vi "Test Raw PubSub.vi"() -> ()   [LabVIEW 2021]
uses:
  typedef/Publisher Configuration.ctl
  typedef/Subscriber Configuration.ctl
  typedef/Publisher Info.ctl
  f88eec82-93b0-4b73-b241-8ea333a750c0.vi
  3ba9bed8-dd13-4a10-92c8-30b1fa84fb7c.vi
  06d7ed46-2aa9-4a58-a146-244b7cae5bd9.vi
  009ccb22-fdf8-4a9a-a05b-4c49a602eecd.vi
  336a4bb3-c987-4874-ab49-fbc20b376376.vi
  d958d2fb-f6ac-4309-8ce0-3eafaa81bea2.vi
  75a58427-ab38-4537-8b56-a141a3672aa3.vi
  6786380f-354a-4568-8806-a035e3271ed9.vi
  422841d8-307b-4ec0-b2db-fbf3b15355db.vi
  2722b832-a6ed-40a1-94d0-5438662527b8.vi
  4f573ed8-5eea-442c-8954-fd33649ad94d.vi
  96719cce-9db7-4fd0-8c85-b901c094f5f7.vi
  9c36c4f5-fd14-474a-8537-d667d986c500.vi
  37cd7a68-2c72-48bd-8358-2e5ff7ad5fbf.vi
  25405cc9-b883-4350-b671-2b1f334a3515.vi
  af1225cd-10e8-4ded-be35-c9aec92c40b2.vi
  a487f0d3-ed83-4ff6-b1b9-975fbbcad064.vi
  1e4a52af-b425-4bd5-8079-be6529fa9e9c.vi
  d9d8694a-5329-4e50-a2e7-87effcffdca9.vi
  4327a0ae-2f84-4360-8cf5-e48e8584a04f.vi
  8254caa6-6f2b-4011-9217-4a5e3ed42d89.vi
  19e9252e-2146-4d1e-ba58-cc4f3a3c56cb.vi
  863d4d22-9275-487b-b92e-4ed484f7a1b3.vi
  c0f4674b-d7d9-47c2-9242-89a7410a619c.vi
  919f7c05-3ba9-40da-9afe-90bc52095352.vi
  1a02b84e-e0dd-4555-bba6-db125e571599.vi
  b1950baf-a6de-4c07-b8a3-a72aac12c1c1.vi
  ae4bf491-c0b7-44fa-a4a7-8158168e9fc6.vi
  ed865d3e-ab37-4a94-9a8c-dd2836983b09.vi
  5089277c-e4c2-417d-bf61-c3bd261b64ad.vi
  2648f811-d11d-4cf1-8e69-7cf28aed7662.vi
  4d02bc77-4783-49f2-a635-9fdf52d75067.vi
  6650dd4f-c820-41cd-8769-445f0eb68481.vi
  363597ae-3dcd-42a2-ad25-38ce26843048.vi
  43a2abd8-1115-4a6b-bb2f-cda109865661.vi
  76c65e38-25cb-4c5d-9514-de54a11eb46c.vi
  076b9f91-9c98-45bc-8a99-05568dd34c74.vi
  da7c517f-bb6b-476f-8057-eaeaf84c1734.vi
  75a22d6a-3c1f-452c-a0ab-9f852fbcf576.vi
  d28d170c-9ca3-4356-a02f-9b2902eae1eb.vi
  458cc294-3f79-4518-a0de-1932c661e4d9.vi
  4369ee51-5961-4433-b656-85aa5b427ae6.vi
  cfff3f0f-7213-4192-9fc9-75e3c3355763.vi
  39bd5219-0461-483e-bfc5-6ac24da31237.vi
  c31ef992-ca3f-413b-a618-0d329516adf2.vi
  e3428d73-0891-455a-b634-5f02aa550c64.vi
  c128d40d-42b3-4721-be74-df15ce752ec7.vi
  SubVIs/Get Path.vi
  SubVIs/Convert Error.vi
  f88eec82-93b0-4b73-b241-8ea333a750c0.vi/f164bb55-fadc-406a-97d8-e3295a396b46.vi
  SubVIs/Add Error.vi
  Refnum/Raw Publisher to Refnum.vi
  <vilib>/CIF Foundation/CIF Utilities/File/File/File Not Found Error Update.vi
  3ba9bed8-dd13-4a10-92c8-30b1fa84fb7c.vi/15451e88-64ef-462d-9cc0-58968935b893.vi
  Refnum/Raw Subscriber to Refnum.vi
  Refnum/Raw Publisher from Refnum.vi
  Refnum/Raw Subscriber from Refnum.vi
  336a4bb3-c987-4874-ab49-fbc20b376376.vi/f164bb55-fadc-406a-97d8-e3295a396b46.vi
  d958d2fb-f6ac-4309-8ce0-3eafaa81bea2.vi/15451e88-64ef-462d-9cc0-58968935b893.vi
  75a58427-ab38-4537-8b56-a141a3672aa3.vi/15451e88-64ef-462d-9cc0-58968935b893.vi
  4f573ed8-5eea-442c-8954-fd33649ad94d.vi/f164bb55-fadc-406a-97d8-e3295a396b46.vi
  96719cce-9db7-4fd0-8c85-b901c094f5f7.vi/15451e88-64ef-462d-9cc0-58968935b893.vi
  9c36c4f5-fd14-474a-8537-d667d986c500.vi/15451e88-64ef-462d-9cc0-58968935b893.vi
  a487f0d3-ed83-4ff6-b1b9-975fbbcad064.vi/f164bb55-fadc-406a-97d8-e3295a396b46.vi
  1e4a52af-b425-4bd5-8079-be6529fa9e9c.vi/15451e88-64ef-462d-9cc0-58968935b893.vi
  d9d8694a-5329-4e50-a2e7-87effcffdca9.vi/15451e88-64ef-462d-9cc0-58968935b893.vi
  863d4d22-9275-487b-b92e-4ed484f7a1b3.vi/f164bb55-fadc-406a-97d8-e3295a396b46.vi
  c0f4674b-d7d9-47c2-9242-89a7410a619c.vi/15451e88-64ef-462d-9cc0-58968935b893.vi
  919f7c05-3ba9-40da-9afe-90bc52095352.vi/15451e88-64ef-462d-9cc0-58968935b893.vi
  1a02b84e-e0dd-4555-bba6-db125e571599.vi/f164bb55-fadc-406a-97d8-e3295a396b46.vi
  ae4bf491-c0b7-44fa-a4a7-8158168e9fc6.vi/15451e88-64ef-462d-9cc0-58968935b893.vi
  5089277c-e4c2-417d-bf61-c3bd261b64ad.vi/f164bb55-fadc-406a-97d8-e3295a396b46.vi
  4d02bc77-4783-49f2-a635-9fdf52d75067.vi/15451e88-64ef-462d-9cc0-58968935b893.vi
  43a2abd8-1115-4a6b-bb2f-cda109865661.vi/f164bb55-fadc-406a-97d8-e3295a396b46.vi
  76c65e38-25cb-4c5d-9514-de54a11eb46c.vi/15451e88-64ef-462d-9cc0-58968935b893.vi
  458cc294-3f79-4518-a0de-1932c661e4d9.vi/f164bb55-fadc-406a-97d8-e3295a396b46.vi
  4369ee51-5961-4433-b656-85aa5b427ae6.vi/15451e88-64ef-462d-9cc0-58968935b893.vi
  c128d40d-42b3-4721-be74-df15ce752ec7.vi/f164bb55-fadc-406a-97d8-e3295a396b46.vi
  <vilib>/Utility/error.llb/Trim Whitespace.vi
  SubVIs/Add Error Core.vi
  <vilib>/CIF Foundation/CIF Utilities/DataTypes/Utilities/Get Element Info of Variant.vi
  SubVIs/Get Type String.vi
  <vilib>/CIF Foundation/CIF Utilities/DataTypes/Utilities/Get JSON Descriptor of Variant.vi
  SubVIs/Convert Error Core.vi
  <vilib>/CIF Foundation/CIF Utilities/File/SubVIs/File Not Found Error Core.vi
  Iceoryx.lvlib
panel:
  out "status":string
  out "pass":bool
  out "error out":errorcluster
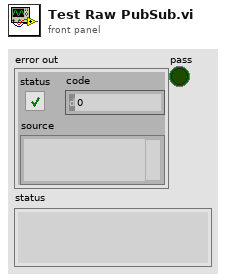
[diagram p1: front panel]
types:
  T1 = typedef "Iceoryx.lvlib/Subscriber Configuration.ctl" = cluster{"Name":string, "Topic":string, "Type":string, "Backpressure":bool}
  T2 = typedef "Iceoryx.lvlib/Publisher Configuration.ctl" = cluster{"Name":string, "Topic":string, "Type":string, "Best Effort Subscribers":u32, "Backpressure Subscribers":u32, "Best Effort Queue Depth":u32, "Backpressure Queue Depth":u32}
  T3 = typedef "Iceoryx.lvlib/Publisher Info.ctl" = cluster{"Type":string, "Element Size":u32, "Max Elements in Array":u32, "Backpressure Queue Depth":u32, "Best Effort Queue Depth":u32}
  T4 = typedef "Iceoryx.lvlib/Raw Publisher Refnum.ctl" = cluster{"refnum":u64, "Raw Pub":enum8{"rawpub"}}
  T5 = typedef "Iceoryx.lvlib/Raw Subscriber Refnum.ctl" = cluster{"refnum":u64, "Raw Sub":enum8{"rawsub"}}
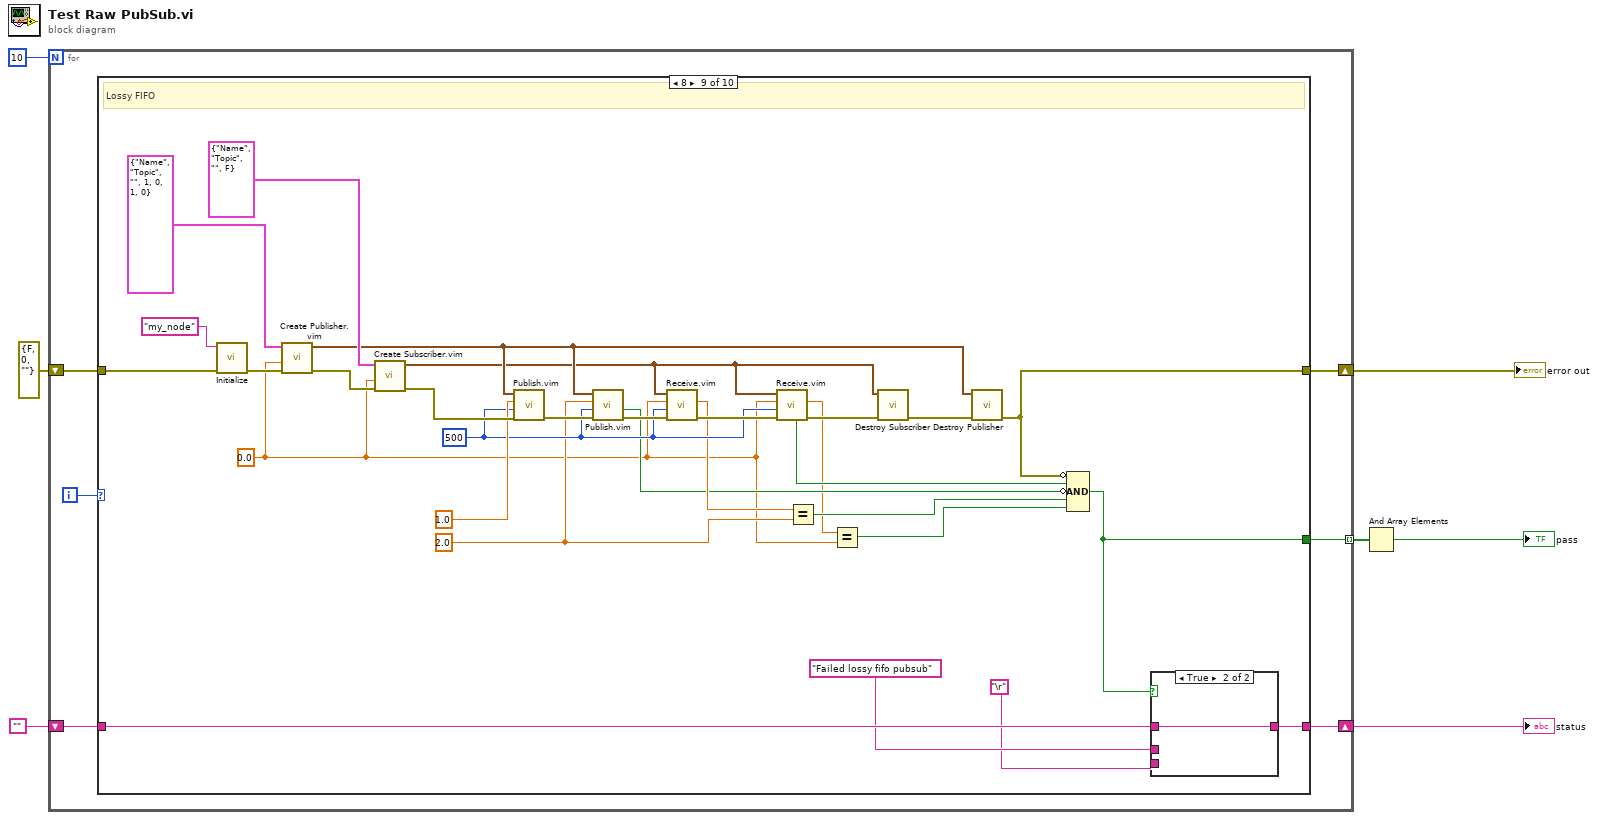
[diagram p0: block diagram]
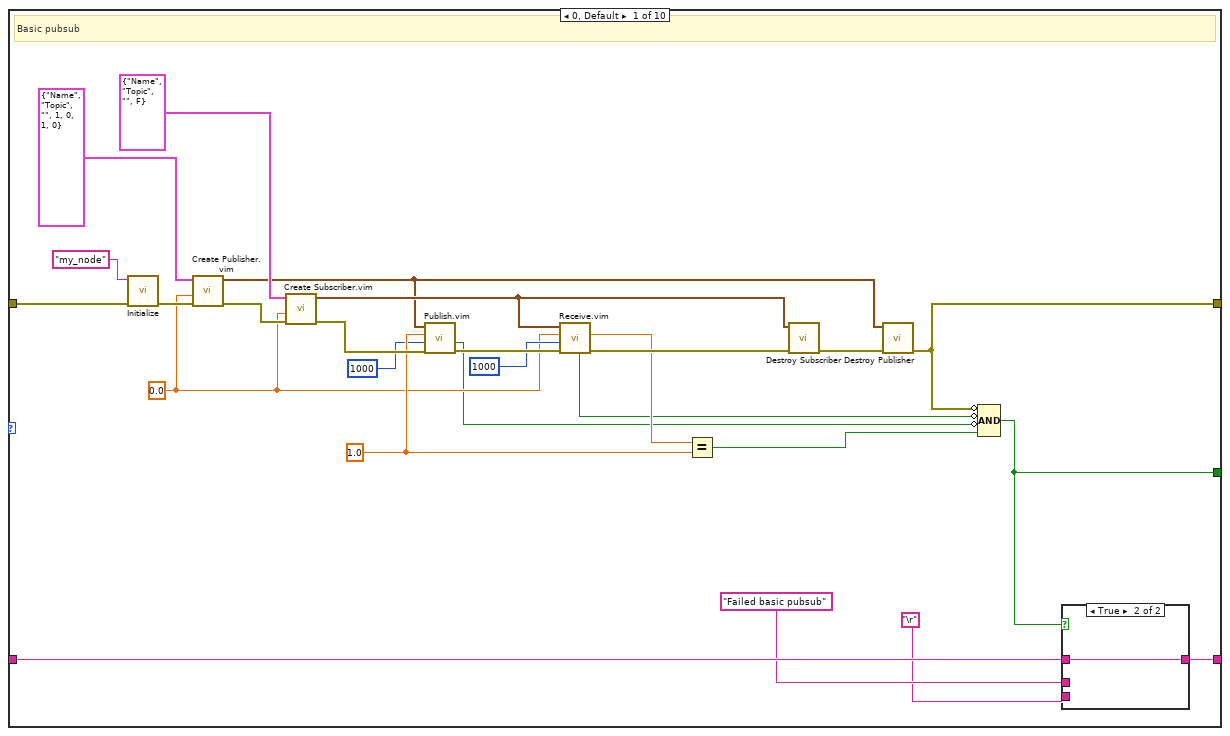
[diagram p2: hidden frame]
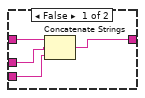
[diagram p3: hidden frame]
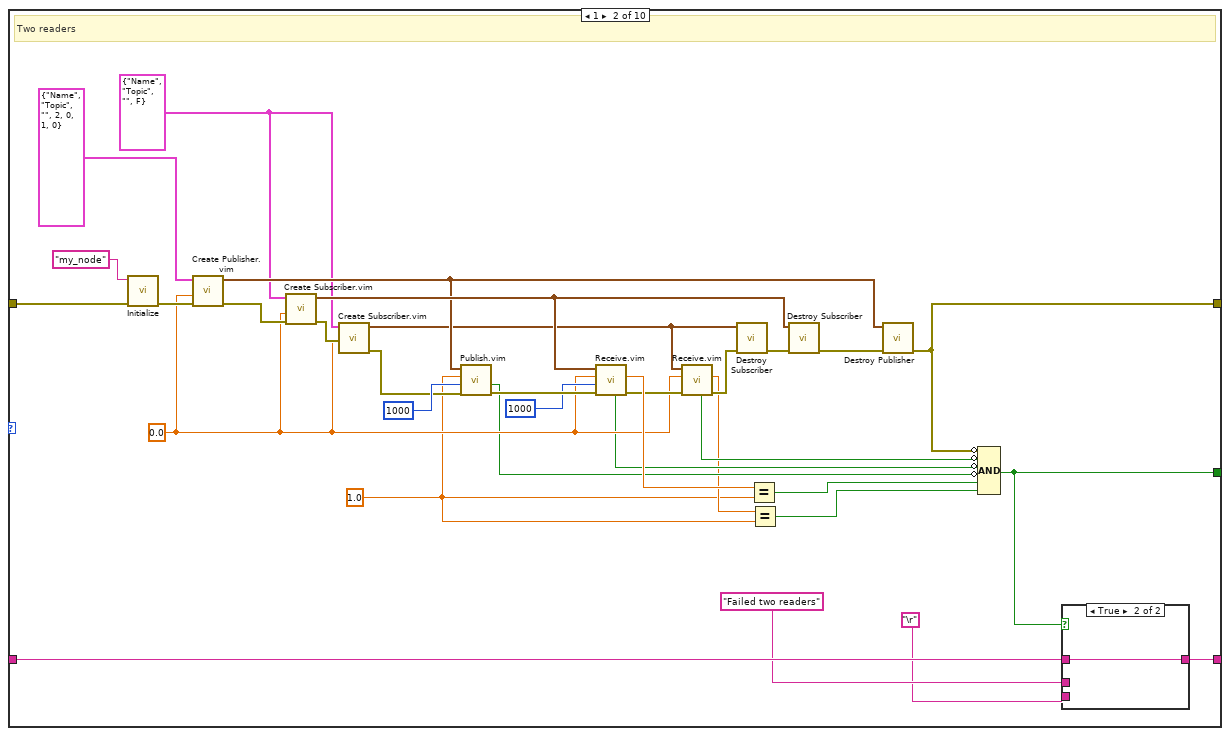
[diagram p4: hidden frame]
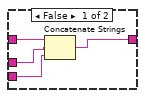
[diagram p5: hidden frame]
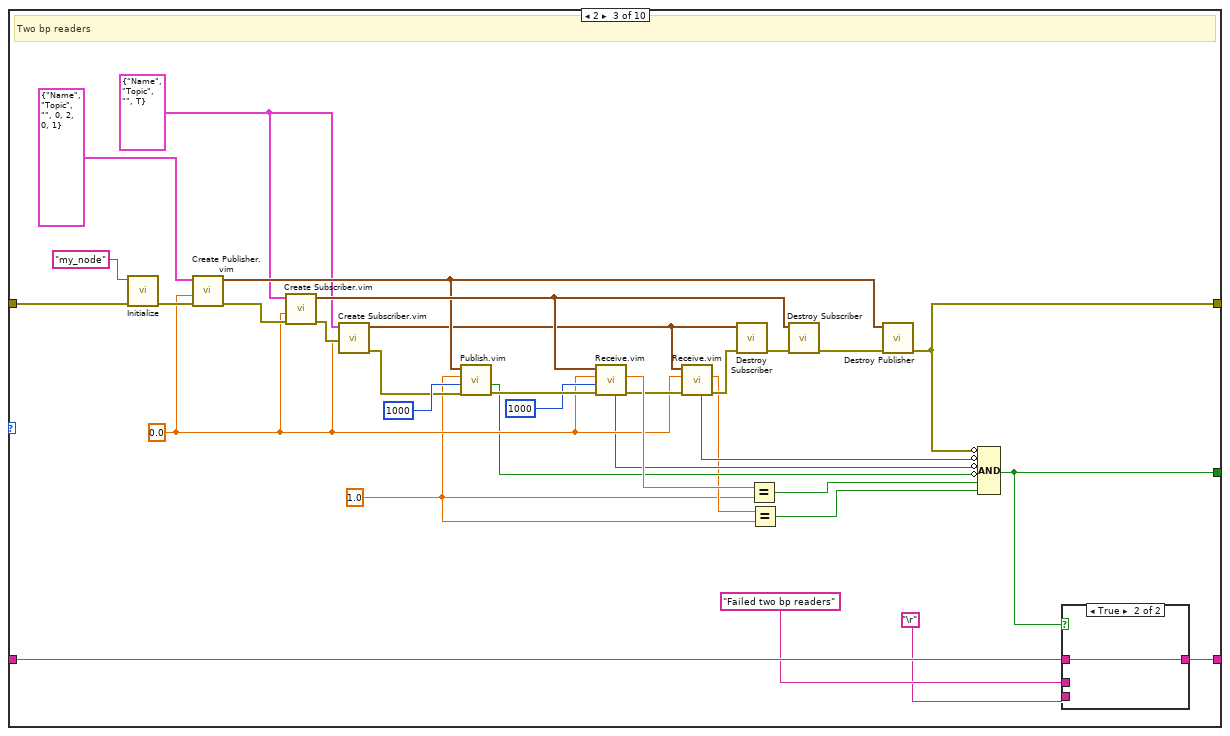
[diagram p6: hidden frame]
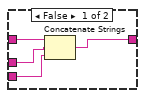
[diagram p7: hidden frame]
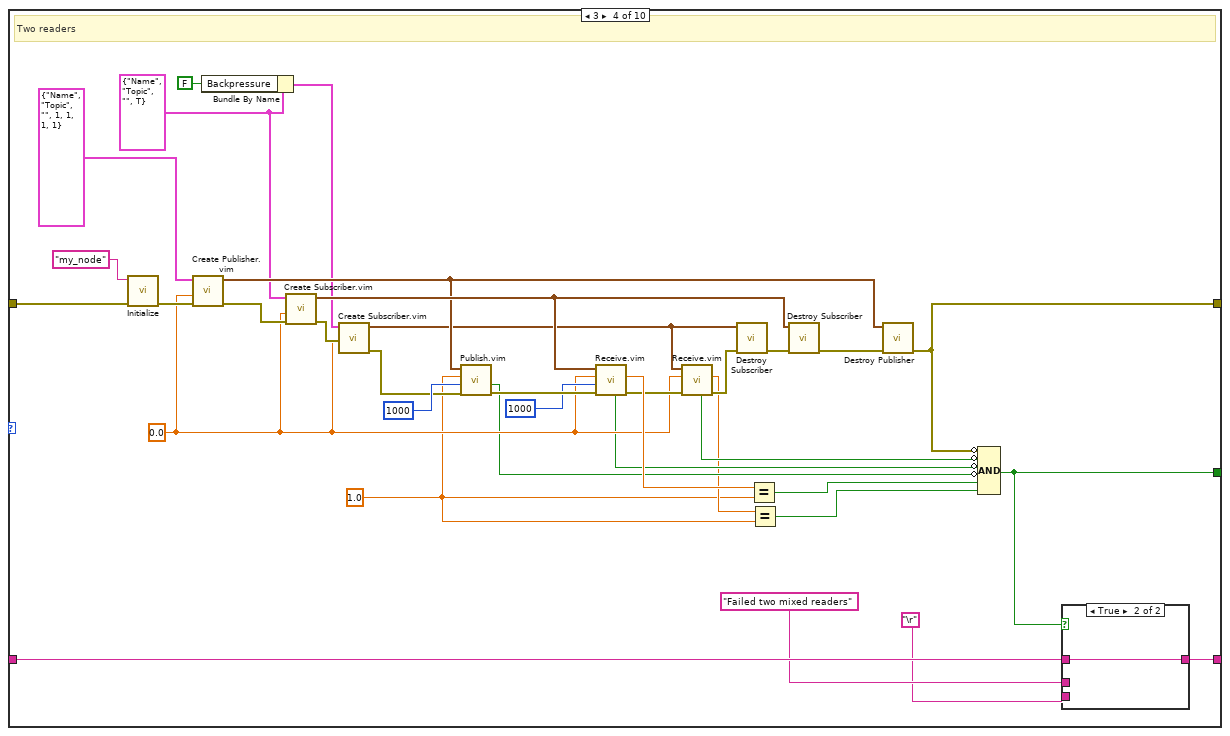
[diagram p8: hidden frame]
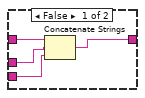
[diagram p9: hidden frame]
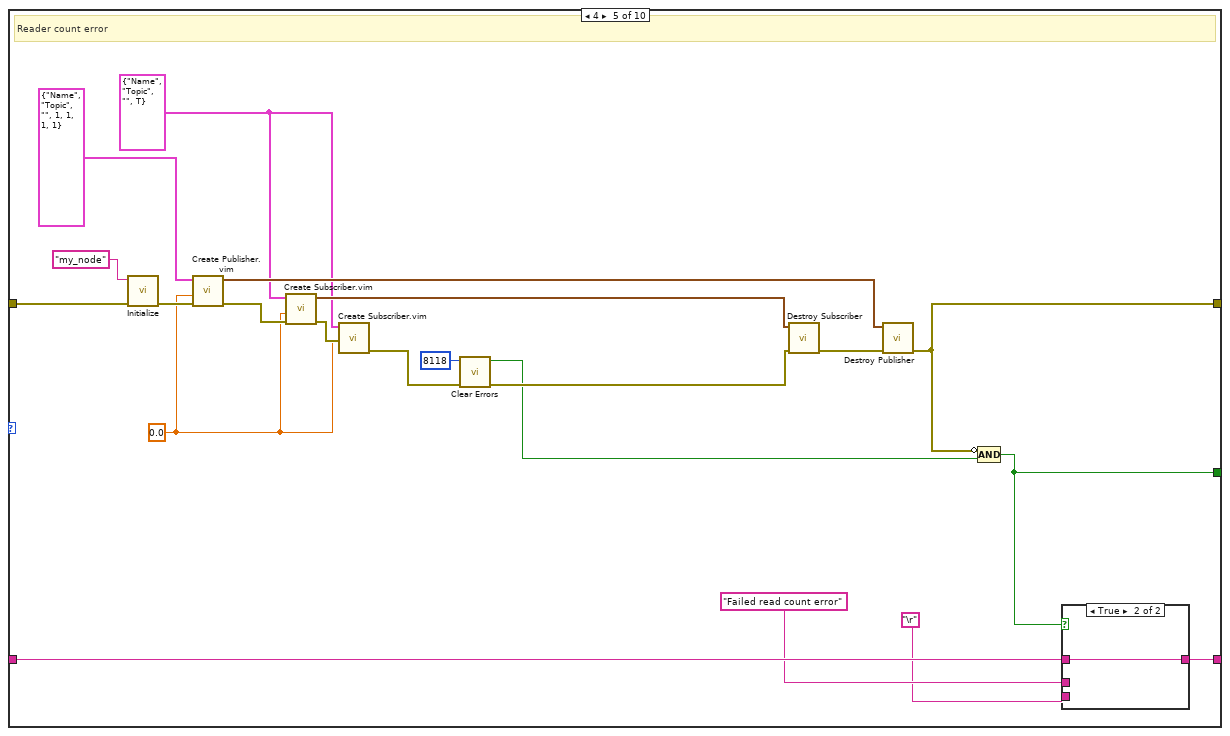
[diagram p10: hidden frame]
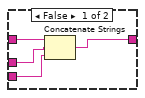
[diagram p11: hidden frame]
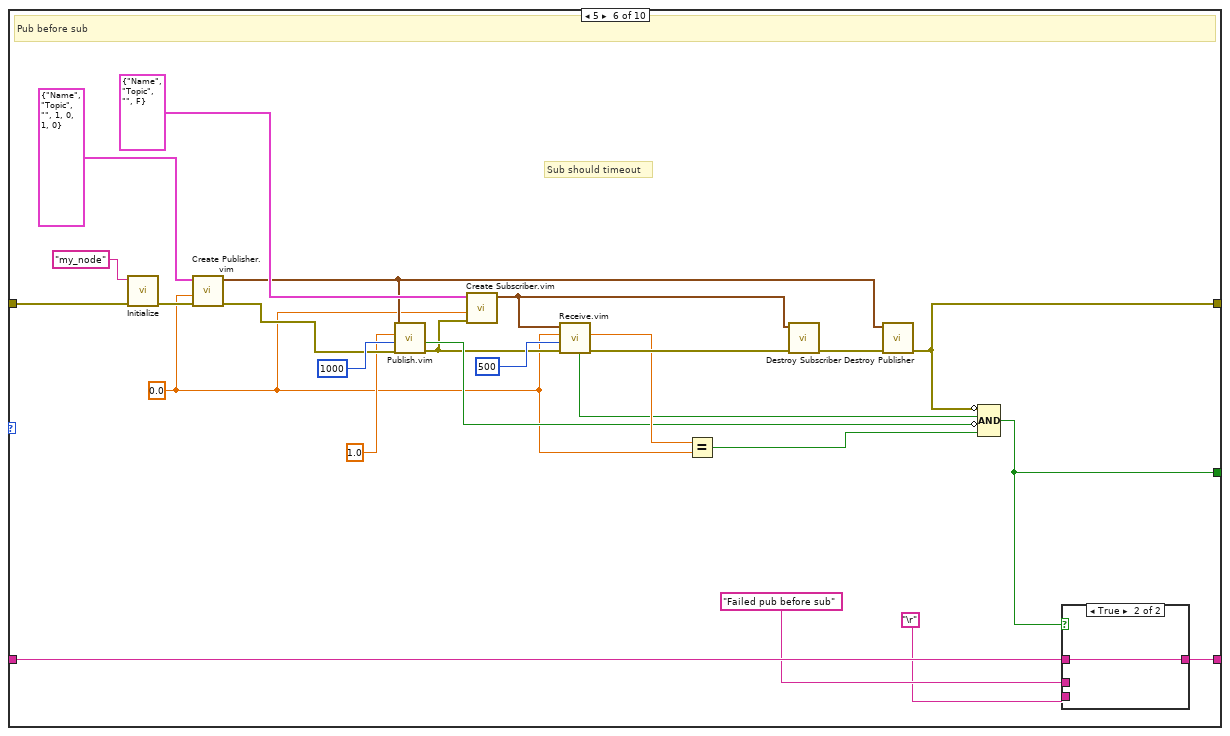
[diagram p12: hidden frame]
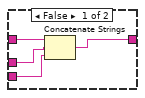
[diagram p13: hidden frame]
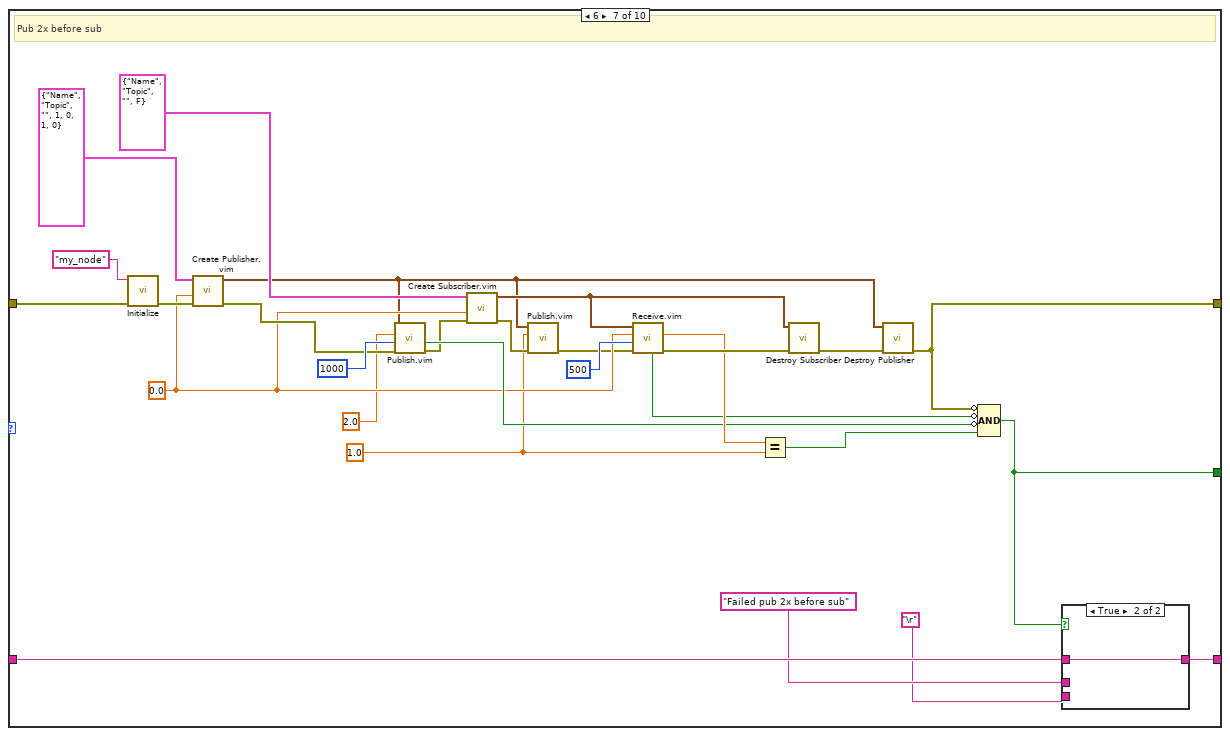
[diagram p14: hidden frame]
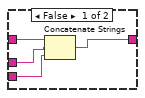
[diagram p15: hidden frame]
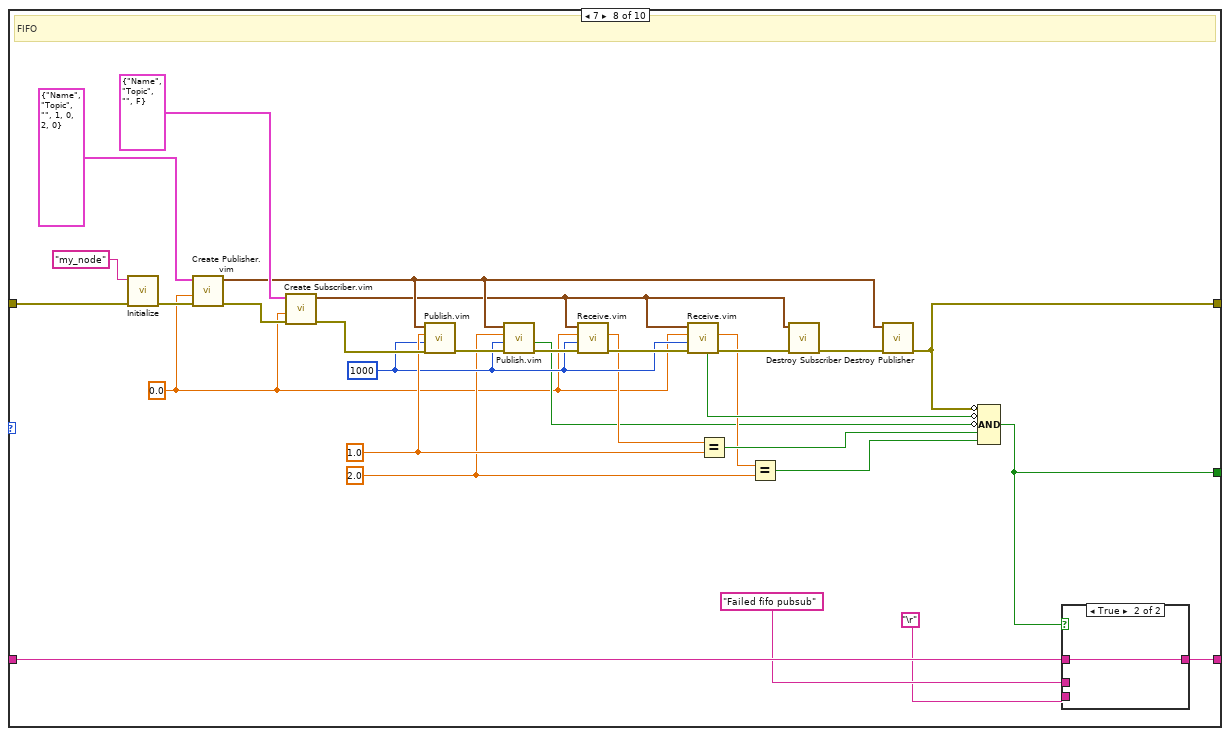
[diagram p16: hidden frame]
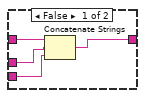
[diagram p17: hidden frame]
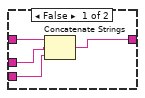
[diagram p18: hidden frame]
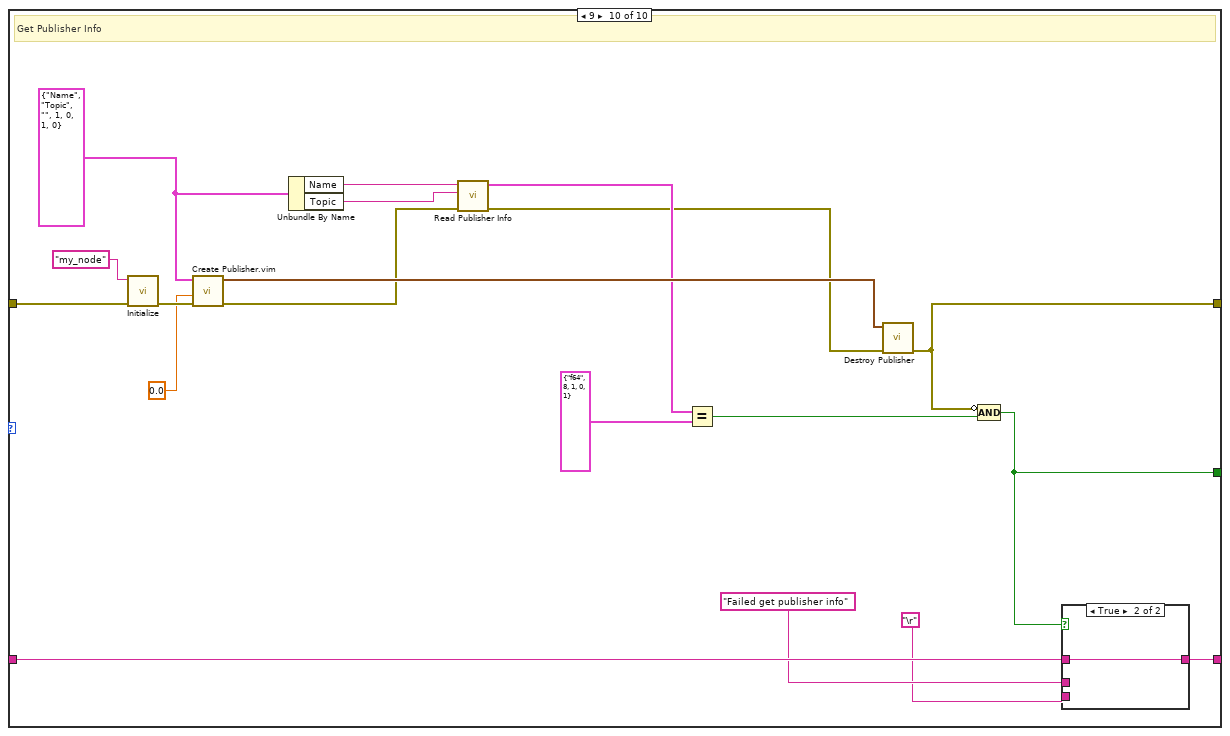
[diagram p19: hidden frame]
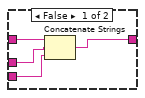
[diagram p20: hidden frame]
diagram:
  n1 = for {
    N: 10 -> [_]
    tunnel: [w13] -> w7 mode=indexing
    shift-right: [w10] -> w3
    shift-left: "" -> [w11]
    shift-right: [w9] -> w1
    shift-left: errorcluster {"status"=FALSE, "code"=0, "source"=""} ("error out") -> [w8]
    i -> [w12]
    n2 = case shown="8" w12 {
      tunnel: [w35 w73 w111 w151 w177 w207 w240 w275 w310 w334] -> w13
      tunnel: w11 -> [w39 w77 w115 w155 w181 w211 w244 w279 w314 w338]
      tunnel: [w38 w76 w114 w154 w180 w210 w243 w278 w313 w337] -> w10
      tunnel: [w22 w63 w101 w141 w168 w197 w231 w265 w300 w329] -> w9
      tunnel: w8 -> [w34 w72 w110 w150 w176 w206 w239 w274 w309 w333]
      frame 0, Default {
        w18 = 0.0
        w21 = 1.0
        # "Basic pubsub"
        n3 = call "Initialize.vi"("error in (no error)"=w34, "Node name"="my_node") -> ("error out"=w30:errorcluster)  [unwired: 9 in]
        n4 = call "Create Publisher.vim"("error in (no error)"=w30, "Data"=w18, "Publisher Configuration"=T2 {"Name"="Name", "Topic"="Topic", "Type"="", "Best Effort Subscribers"=1, "Backpressure Subscribers"=0, "Best Effort Queue Depth"=1, "Backpressure Queue Depth"=0}) -> ("error out"=w29:errorcluster, "Publisher Reference"=w23:T4)  [unwired: 6 in, 1 out]
        n5 = call "Create Subscriber.vim"("error in (no error)"=w29, "Data Type"=w18, "Subscriber Configuration"=T1 {"Name"="Name", "Topic"="Topic", "Type"="", "Backpressure"=FALSE}) -> ("error out"=w28:errorcluster, "Subscriber Reference"=w25:T5)  [unwired: 6 in, 1 out]
        n6 = call "Publish.vim"("error in (no error)"=w28, "Timoeut ms"=u32 1000, "Data In"=w21, "Publisher Reference"=w23) -> ("error out"=w27:errorcluster, "Timeout"=w15:bool)  [unwired: 5 in, 1 out]
        n7 = call "Receive.vim"("error in (no error)"=w27, "Timoeut ms"=u32 1000, "Data In"=w18, "Subscriber Reference"=w25) -> ("error out"=w26:errorcluster, "Data Out"=w17:dbl, "Timeout"=w14:bool)  [unwired: 4 in, 1 out]
        n8 = Equal?(x=w17, y=w21) -> (x = y?=w16:bool)
        n9 = call "Destroy Subscriber.vi"("error in (no error)"=w26, "Subscriber Reference"=w25) -> ("error out"=w24:errorcluster)  [unwired: 9 in]
        n10 = call "Destroy Publisher.vi"("error in (no error)"=w24, "Publisher Reference"=w23) -> ("error out"=w22:errorcluster)  [unwired: 9 in]
        n11 = Compound Arithmetic op=AND(invert w22, invert w14, invert w15, w16) -> (w35:bool)
        n12 = case shown="True" w35 {
          tunnel: w39 -> [w43 w44]
          tunnel: [w40 w44] -> w38
          tunnel: "Failed basic pubsub" -> [w42 _]
          tunnel: "\r" -> [w41 _]
          frame False {
            n13 = Concatenate Strings(w43, w42, w41) -> (w40:string)
          }
          frame True {
          }
        }
      }
      frame 1 {
        w57 = T1 {"Name"="Name", "Topic"="Topic", "Type"="", "Backpressure"=FALSE} ("Subscriber Configuration")
        w52 = 0.0
        w47 = 1.0
        # "Two readers"
        n14 = call "Initialize.vi"("error in (no error)"=w72, "Node name"="my_node") -> ("error out"=w69:errorcluster)  [unwired: 9 in]
        n15 = call "Create Publisher.vim"("error in (no error)"=w69, "Data"=w52, "Publisher Configuration"=T2 {"Name"="Name", "Topic"="Topic", "Type"="", "Best Effort Subscribers"=2, "Backpressure Subscribers"=0, "Best Effort Queue Depth"=1, "Backpressure Queue Depth"=0}) -> ("error out"=w68:errorcluster, "Publisher Reference"=w64:T4)  [unwired: 6 in, 1 out]
        n16 = call "Create Subscriber.vim"("error in (no error)"=w68, "Data Type"=w52, "Subscriber Configuration"=w57) -> ("error out"=w59:errorcluster, "Subscriber Reference"=w66:T5)  [unwired: 6 in, 1 out]
        n17 = call "Create Subscriber.vim"("error in (no error)"=w59, "Data Type"=w52, "Subscriber Configuration"=w57) -> ("error out"=w58:errorcluster, "Subscriber Reference"=w53:T5)  [unwired: 6 in, 1 out]
        n18 = call "Publish.vim"("error in (no error)"=w58, "Timoeut ms"=u32 1000, "Data In"=w47, "Publisher Reference"=w64) -> ("error out"=w67:errorcluster, "Timeout"=w51:bool)  [unwired: 5 in, 1 out]
        n19 = call "Receive.vim"("error in (no error)"=w67, "Timoeut ms"=u32 1000, "Data In"=w52, "Subscriber Reference"=w66) -> ("error out"=w56:errorcluster, "Data Out"=w60:dbl, "Timeout"=w50:bool)  [unwired: 4 in, 1 out]
        n20 = call "Receive.vim"("error in (no error)"=w56, "Data In"=w52, "Subscriber Reference"=w53) -> ("error out"=w55:errorcluster, "Data Out"=w48:dbl, "Timeout"=w49:bool)  [unwired: 5 in, 1 out]
        n21 = call "Destroy Subscriber.vi"("error in (no error)"=w55, "Subscriber Reference"=w53) -> ("error out"=w54:errorcluster)  [unwired: 9 in]
        n22 = Equal?(x=w60, y=w47) -> (x = y?=w46:bool)
        n23 = Equal?(x=w48, y=w47) -> (x = y?=w45:bool)
        n24 = call "Destroy Subscriber.vi"("error in (no error)"=w54, "Subscriber Reference"=w66) -> ("error out"=w65:errorcluster)  [unwired: 9 in]
        n25 = call "Destroy Publisher.vi"("error in (no error)"=w65, "Publisher Reference"=w64) -> ("error out"=w63:errorcluster)  [unwired: 9 in]
        n26 = Compound Arithmetic op=AND(invert w63, invert w49, invert w50, invert w51, w46, w45) -> (w73:bool)
        n27 = case shown="True" w73 {
          tunnel: w77 -> [w81 w82]
          tunnel: [w78 w82] -> w76
          tunnel: "Failed two readers" -> [w80 _]
          tunnel: "\r" -> [w79 _]
          frame False {
            n28 = Concatenate Strings(w81, w80, w79) -> (w78:string)
          }
          frame True {
          }
        }
      }
      frame 2 {
        w95 = T1 {"Name"="Name", "Topic"="Topic", "Type"="", "Backpressure"=TRUE} ("Subscriber Configuration")
        w90 = 0.0
        w85 = 1.0
        # "Two bp readers"
        n29 = call "Initialize.vi"("error in (no error)"=w110, "Node name"="my_node") -> ("error out"=w107:errorcluster)  [unwired: 9 in]
        n30 = call "Create Publisher.vim"("error in (no error)"=w107, "Data"=w90, "Publisher Configuration"=T2 {"Name"="Name", "Topic"="Topic", "Type"="", "Best Effort Subscribers"=0, "Backpressure Subscribers"=2, "Best Effort Queue Depth"=0, "Backpressure Queue Depth"=1}) -> ("error out"=w106:errorcluster, "Publisher Reference"=w102:T4)  [unwired: 6 in, 1 out]
        n31 = call "Create Subscriber.vim"("error in (no error)"=w106, "Data Type"=w90, "Subscriber Configuration"=w95) -> ("error out"=w97:errorcluster, "Subscriber Reference"=w104:T5)  [unwired: 6 in, 1 out]
        n32 = call "Create Subscriber.vim"("error in (no error)"=w97, "Data Type"=w90, "Subscriber Configuration"=w95) -> ("error out"=w96:errorcluster, "Subscriber Reference"=w91:T5)  [unwired: 6 in, 1 out]
        n33 = call "Publish.vim"("error in (no error)"=w96, "Timoeut ms"=u32 1000, "Data In"=w85, "Publisher Reference"=w102) -> ("error out"=w105:errorcluster, "Timeout"=w89:bool)  [unwired: 5 in, 1 out]
        n34 = call "Receive.vim"("error in (no error)"=w105, "Timoeut ms"=u32 1000, "Data In"=w90, "Subscriber Reference"=w104) -> ("error out"=w94:errorcluster, "Data Out"=w98:dbl, "Timeout"=w88:bool)  [unwired: 4 in, 1 out]
        n35 = call "Receive.vim"("error in (no error)"=w94, "Data In"=w90, "Subscriber Reference"=w91) -> ("error out"=w93:errorcluster, "Data Out"=w86:dbl, "Timeout"=w87:bool)  [unwired: 5 in, 1 out]
        n36 = call "Destroy Subscriber.vi"("error in (no error)"=w93, "Subscriber Reference"=w91) -> ("error out"=w92:errorcluster)  [unwired: 9 in]
        n37 = Equal?(x=w98, y=w85) -> (x = y?=w84:bool)
        n38 = Equal?(x=w86, y=w85) -> (x = y?=w83:bool)
        n39 = call "Destroy Subscriber.vi"("error in (no error)"=w92, "Subscriber Reference"=w104) -> ("error out"=w103:errorcluster)  [unwired: 9 in]
        n40 = call "Destroy Publisher.vi"("error in (no error)"=w103, "Publisher Reference"=w102) -> ("error out"=w101:errorcluster)  [unwired: 9 in]
        n41 = Compound Arithmetic op=AND(invert w101, invert w87, invert w88, invert w89, w84, w83) -> (w111:bool)
        n42 = case shown="True" w111 {
          tunnel: w115 -> [w119 w120]
          tunnel: [w116 w120] -> w114
          tunnel: "Failed two bp readers" -> [w118 _]
          tunnel: "\r" -> [w117 _]
          frame False {
            n43 = Concatenate Strings(w119, w118, w117) -> (w116:string)
          }
          frame True {
          }
        }
      }
      frame 3 {
        w123 = T1 {"Name"="Name", "Topic"="Topic", "Type"="", "Backpressure"=TRUE} ("Subscriber Configuration")
        w131 = 0.0
        w126 = 1.0
        # "Two readers"
        n44 = call "Initialize.vi"("error in (no error)"=w150, "Node name"="my_node") -> ("error out"=w147:errorcluster)  [unwired: 9 in]
        n45 = call "Create Publisher.vim"("error in (no error)"=w147, "Data"=w131, "Publisher Configuration"=T2 {"Name"="Name", "Topic"="Topic", "Type"="", "Best Effort Subscribers"=1, "Backpressure Subscribers"=1, "Best Effort Queue Depth"=1, "Backpressure Queue Depth"=1}) -> ("error out"=w146:errorcluster, "Publisher Reference"=w142:T4)  [unwired: 6 in, 1 out]
        n46 = Bundle By Name(cluster=w123, "Backpressure"=FALSE) -> (w121:T1)
        n47 = call "Create Subscriber.vim"("error in (no error)"=w146, "Data Type"=w131, "Subscriber Configuration"=w123) -> ("error out"=w137:errorcluster, "Subscriber Reference"=w144:T5)  [unwired: 6 in, 1 out]
        n48 = call "Create Subscriber.vim"("error in (no error)"=w137, "Data Type"=w131, "Subscriber Configuration"=w121) -> ("error out"=w136:errorcluster, "Subscriber Reference"=w132:T5)  [unwired: 6 in, 1 out]
        n49 = call "Publish.vim"("error in (no error)"=w136, "Timoeut ms"=u32 1000, "Data In"=w126, "Publisher Reference"=w142) -> ("error out"=w145:errorcluster, "Timeout"=w130:bool)  [unwired: 5 in, 1 out]
        n50 = call "Receive.vim"("error in (no error)"=w145, "Timoeut ms"=u32 1000, "Data In"=w131, "Subscriber Reference"=w144) -> ("error out"=w135:errorcluster, "Data Out"=w138:dbl, "Timeout"=w129:bool)  [unwired: 4 in, 1 out]
        n51 = call "Receive.vim"("error in (no error)"=w135, "Data In"=w131, "Subscriber Reference"=w132) -> ("error out"=w134:errorcluster, "Data Out"=w127:dbl, "Timeout"=w128:bool)  [unwired: 5 in, 1 out]
        n52 = call "Destroy Subscriber.vi"("error in (no error)"=w134, "Subscriber Reference"=w132) -> ("error out"=w133:errorcluster)  [unwired: 9 in]
        n53 = Equal?(x=w138, y=w126) -> (x = y?=w125:bool)
        n54 = Equal?(x=w127, y=w126) -> (x = y?=w124:bool)
        n55 = call "Destroy Subscriber.vi"("error in (no error)"=w133, "Subscriber Reference"=w144) -> ("error out"=w143:errorcluster)  [unwired: 9 in]
        n56 = call "Destroy Publisher.vi"("error in (no error)"=w143, "Publisher Reference"=w142) -> ("error out"=w141:errorcluster)  [unwired: 9 in]
        n57 = Compound Arithmetic op=AND(invert w141, invert w128, invert w129, invert w130, w125, w124) -> (w151:bool)
        n58 = case shown="True" w151 {
          tunnel: w155 -> [w159 w160]
          tunnel: [w156 w160] -> w154
          tunnel: "Failed two mixed readers" -> [w158 _]
          tunnel: "\r" -> [w157 _]
          frame False {
            n59 = Concatenate Strings(w159, w158, w157) -> (w156:string)
          }
          frame True {
          }
        }
      }
      frame 4 {
        w165 = T1 {"Name"="Name", "Topic"="Topic", "Type"="", "Backpressure"=TRUE} ("Subscriber Configuration")
        w166 = 0.0
        # "Reader count error"
        n60 = call "Initialize.vi"("error in (no error)"=w176, "Node name"="my_node") -> ("error out"=w173:errorcluster)  [unwired: 9 in]
        n61 = call "Create Publisher.vim"("error in (no error)"=w173, "Data"=w166, "Publisher Configuration"=T2 {"Name"="Name", "Topic"="Topic", "Type"="", "Best Effort Subscribers"=1, "Backpressure Subscribers"=1, "Best Effort Queue Depth"=1, "Backpressure Queue Depth"=1}) -> ("error out"=w172:errorcluster, "Publisher Reference"=w169:T4)  [unwired: 6 in, 1 out]
        n62 = call "Create Subscriber.vim"("error in (no error)"=w172, "Data Type"=w166, "Subscriber Configuration"=w165) -> ("error out"=w167:errorcluster, "Subscriber Reference"=w171:T5)  [unwired: 6 in, 1 out]
        n63 = call "Create Subscriber.vim"("error in (no error)"=w167, "Data Type"=w166, "Subscriber Configuration"=w165) -> ("error out"=w164:errorcluster)  [unwired: 6 in, 2 out]
        n64 = call <vilib>:"Clear Errors.vi"("error in (no error)"=w164, "specific error code to clear (0: all)"=8118) -> ("error out"=w162:errorcluster, "specific error cleared?"=w161:bool)  [unwired: 4 in]
        n65 = call "Destroy Subscriber.vi"("error in (no error)"=w162, "Subscriber Reference"=w171) -> ("error out"=w170:errorcluster)  [unwired: 9 in]
        n66 = call "Destroy Publisher.vi"("error in (no error)"=w170, "Publisher Reference"=w169) -> ("error out"=w168:errorcluster)  [unwired: 9 in]
        n67 = Compound Arithmetic op=AND(invert w168, w161) -> (w177:bool)
        n68 = case shown="True" w177 {
          tunnel: w181 -> [w185 w186]
          tunnel: [w182 w186] -> w180
          tunnel: "Failed read count error" -> [w184 _]
          tunnel: "\r" -> [w183 _]
          frame False {
            n69 = Concatenate Strings(w185, w184, w183) -> (w182:string)
          }
          frame True {
          }
        }
      }
      frame 5 {
        w187 = 0.0
        # "Sub should timeout"
        # "Pub before sub"
        n70 = call "Initialize.vi"("error in (no error)"=w206, "Node name"="my_node") -> ("error out"=w202:errorcluster)  [unwired: 9 in]
        n71 = call "Create Publisher.vim"("error in (no error)"=w202, "Data"=w187, "Publisher Configuration"=T2 {"Name"="Name", "Topic"="Topic", "Type"="", "Best Effort Subscribers"=1, "Backpressure Subscribers"=0, "Best Effort Queue Depth"=1, "Backpressure Queue Depth"=0}) -> ("error out"=w189:errorcluster, "Publisher Reference"=w198:T4)  [unwired: 6 in, 1 out]
        n72 = call "Publish.vim"("error in (no error)"=w189, "Timoeut ms"=u32 1000, "Data In"=1.0, "Publisher Reference"=w198) -> ("error out"=w190:errorcluster, "Timeout"=w192:bool)  [unwired: 5 in, 1 out]
        n73 = call "Create Subscriber.vim"("error in (no error)"=w190, "Data Type"=w187, "Subscriber Configuration"=T1 {"Name"="Name", "Topic"="Topic", "Type"="", "Backpressure"=FALSE}) -> ("Subscriber Reference"=w200:T5)  [unwired: 6 in, 2 out]
        n74 = call "Receive.vim"("error in (no error)"=w190, "Timoeut ms"=u32 500, "Data In"=w187, "Subscriber Reference"=w200) -> ("error out"=w201:errorcluster, "Data Out"=w194:dbl, "Timeout"=w191:bool)  [unwired: 4 in, 1 out]
        n75 = Equal?(x=w194, y=w187) -> (x = y?=w193:bool)
        n76 = call "Destroy Subscriber.vi"("error in (no error)"=w201, "Subscriber Reference"=w200) -> ("error out"=w199:errorcluster)  [unwired: 9 in]
        n77 = call "Destroy Publisher.vi"("error in (no error)"=w199, "Publisher Reference"=w198) -> ("error out"=w197:errorcluster)  [unwired: 9 in]
        n78 = Compound Arithmetic op=AND(invert w197, w191, invert w192, w193) -> (w207:bool)
        n79 = case shown="True" w207 {
          tunnel: w211 -> [w215 w216]
          tunnel: [w212 w216] -> w210
          tunnel: "Failed pub before sub" -> [w214 _]
          tunnel: "\r" -> [w213 _]
          frame False {
            n80 = Concatenate Strings(w215, w214, w213) -> (w212:string)
          }
          frame True {
          }
        }
      }
      frame 6 {
        w223 = 0.0
        w217 = 1.0
        # "Pub 2x before sub"
        n81 = call "Initialize.vi"("error in (no error)"=w239, "Node name"="my_node") -> ("error out"=w235:errorcluster)  [unwired: 9 in]
        n82 = call "Create Publisher.vim"("error in (no error)"=w235, "Data"=w223, "Publisher Configuration"=T2 {"Name"="Name", "Topic"="Topic", "Type"="", "Best Effort Subscribers"=1, "Backpressure Subscribers"=0, "Best Effort Queue Depth"=1, "Backpressure Queue Depth"=0}) -> ("error out"=w224:errorcluster, "Publisher Reference"=w219:T4)  [unwired: 6 in, 1 out]
        n83 = call "Publish.vim"("error in (no error)"=w224, "Timoeut ms"=u32 1000, "Data In"=2.0, "Publisher Reference"=w219) -> ("error out"=w222:errorcluster, "Timeout"=w226:bool)  [unwired: 5 in, 1 out]
        n84 = call "Create Subscriber.vim"("error in (no error)"=w222, "Data Type"=w223, "Subscriber Configuration"=T1 {"Name"="Name", "Topic"="Topic", "Type"="", "Backpressure"=FALSE}) -> ("error out"=w220:errorcluster, "Subscriber Reference"=w233:T5)  [unwired: 6 in, 1 out]
        n85 = call "Publish.vim"("error in (no error)"=w220, "Data In"=w217, "Publisher Reference"=w219) -> ("error out"=w221:errorcluster)  [unwired: 6 in, 2 out]
        n86 = call "Receive.vim"("error in (no error)"=w221, "Timoeut ms"=u32 500, "Data In"=w223, "Subscriber Reference"=w233) -> ("error out"=w234:errorcluster, "Data Out"=w228:dbl, "Timeout"=w225:bool)  [unwired: 4 in, 1 out]
        n87 = Equal?(x=w228, y=w217) -> (x = y?=w227:bool)
        n88 = call "Destroy Subscriber.vi"("error in (no error)"=w234, "Subscriber Reference"=w233) -> ("error out"=w232:errorcluster)  [unwired: 9 in]
        n89 = call "Destroy Publisher.vi"("error in (no error)"=w232, "Publisher Reference"=w219) -> ("error out"=w231:errorcluster)  [unwired: 9 in]
        n90 = Compound Arithmetic op=AND(invert w231, invert w225, invert w226, w227) -> (w240:bool)
        n91 = case shown="True" w240 {
          tunnel: w244 -> [w248 w249]
          tunnel: [w245 w249] -> w243
          tunnel: "Failed pub 2x before sub" -> [w247 _]
          tunnel: "\r" -> [w246 _]
          frame False {
            n92 = Concatenate Strings(w248, w247, w246) -> (w245:string)
          }
          frame True {
          }
        }
      }
      frame 7 {
        w254 = 2.0
        w256 = u32 1000 ("Timoeut ms")
        w250 = 0.0
        w264 = 1.0
        # "FIFO"
        n93 = call "Initialize.vi"("error in (no error)"=w274, "Node name"="my_node") -> ("error out"=w270:errorcluster)  [unwired: 9 in]
        n94 = call "Create Publisher.vim"("error in (no error)"=w270, "Data"=w250, "Publisher Configuration"=T2 {"Name"="Name", "Topic"="Topic", "Type"="", "Best Effort Subscribers"=1, "Backpressure Subscribers"=0, "Best Effort Queue Depth"=2, "Backpressure Queue Depth"=0}) -> ("error out"=w269:errorcluster, "Publisher Reference"=w260:T4)  [unwired: 6 in, 1 out]
        n95 = call "Create Subscriber.vim"("error in (no error)"=w269, "Data Type"=w250, "Subscriber Configuration"=T1 {"Name"="Name", "Topic"="Topic", "Type"="", "Backpressure"=FALSE}) -> ("error out"=w268:errorcluster, "Subscriber Reference"=w258:T5)  [unwired: 6 in, 1 out]
        n96 = call "Publish.vim"("error in (no error)"=w268, "Timoeut ms"=w256, "Data In"=w264, "Publisher Reference"=w260) -> ("error out"=w261:errorcluster)  [unwired: 5 in, 2 out]
        n97 = call "Publish.vim"("error in (no error)"=w261, "Timoeut ms"=w256, "Data In"=w254, "Publisher Reference"=w260) -> ("error out"=w259:errorcluster, "Timeout"=w251:bool)  [unwired: 5 in, 1 out]
        n98 = call "Receive.vim"("error in (no error)"=w259, "Timoeut ms"=w256, "Data In"=w250, "Subscriber Reference"=w258) -> ("error out"=w257:errorcluster, "Data Out"=w255:dbl)  [unwired: 4 in, 2 out]
        n99 = call "Receive.vim"("error in (no error)"=w257, "Timoeut ms"=w256, "Data In"=w250, "Subscriber Reference"=w258) -> ("error out"=w267:errorcluster, "Data Out"=w253:dbl, "Timeout"=w262:bool)  [unwired: 4 in, 1 out]
        n100 = Equal?(x=w255, y=w264) -> (x = y?=w263:bool)
        n101 = Equal?(x=w253, y=w254) -> (x = y?=w252:bool)
        n102 = call "Destroy Subscriber.vi"("error in (no error)"=w267, "Subscriber Reference"=w258) -> ("error out"=w266:errorcluster)  [unwired: 9 in]
        n103 = call "Destroy Publisher.vi"("error in (no error)"=w266, "Publisher Reference"=w260) -> ("error out"=w265:errorcluster)  [unwired: 9 in]
        n104 = Compound Arithmetic op=AND(invert w265, invert w262, invert w251, w263, w252) -> (w275:bool)
        n105 = case shown="True" w275 {
          tunnel: w279 -> [w283 w284]
          tunnel: [w280 w284] -> w278
          tunnel: "Failed fifo pubsub" -> [w282 _]
          tunnel: "\r" -> [w281 _]
          frame False {
            n106 = Concatenate Strings(w283, w282, w281) -> (w280:string)
          }
          frame True {
          }
        }
      }
      frame 8 {
        w288 = 2.0
        w291 = u32 500 ("Timoeut ms")
        w286 = 0.0
        # "Lossy FIFO"
        n107 = call "Initialize.vi"("error in (no error)"=w309, "Node name"="my_node") -> ("error out"=w305:errorcluster)  [unwired: 9 in]
        n108 = call "Create Publisher.vim"("error in (no error)"=w305, "Data"=w286, "Publisher Configuration"=T2 {"Name"="Name", "Topic"="Topic", "Type"="", "Best Effort Subscribers"=1, "Backpressure Subscribers"=0, "Best Effort Queue Depth"=1, "Backpressure Queue Depth"=0}) -> ("error out"=w304:errorcluster, "Publisher Reference"=w295:T4)  [unwired: 6 in, 1 out]
        n109 = call "Create Subscriber.vim"("error in (no error)"=w304, "Data Type"=w286, "Subscriber Configuration"=T1 {"Name"="Name", "Topic"="Topic", "Type"="", "Backpressure"=FALSE}) -> ("error out"=w303:errorcluster, "Subscriber Reference"=w293:T5)  [unwired: 6 in, 1 out]
        n110 = call "Publish.vim"("error in (no error)"=w303, "Timoeut ms"=w291, "Data In"=1.0, "Publisher Reference"=w295) -> ("error out"=w296:errorcluster)  [unwired: 5 in, 2 out]
        n111 = call "Publish.vim"("error in (no error)"=w296, "Timoeut ms"=w291, "Data In"=w288, "Publisher Reference"=w295) -> ("error out"=w294:errorcluster, "Timeout"=w289:bool)  [unwired: 5 in, 1 out]
        n112 = call "Receive.vim"("error in (no error)"=w294, "Timoeut ms"=w291, "Data In"=w286, "Subscriber Reference"=w293) -> ("error out"=w292:errorcluster, "Data Out"=w290:dbl)  [unwired: 4 in, 2 out]
        n113 = call "Receive.vim"("error in (no error)"=w292, "Timoeut ms"=w291, "Data In"=w286, "Subscriber Reference"=w293) -> ("error out"=w302:errorcluster, "Data Out"=w287:dbl, "Timeout"=w297:bool)  [unwired: 4 in, 1 out]
        n114 = Equal?(x=w290, y=w288) -> (x = y?=w298:bool)
        n115 = Equal?(x=w287, y=w286) -> (x = y?=w285:bool)
        n116 = call "Destroy Subscriber.vi"("error in (no error)"=w302, "Subscriber Reference"=w293) -> ("error out"=w301:errorcluster)  [unwired: 9 in]
        n117 = call "Destroy Publisher.vi"("error in (no error)"=w301, "Publisher Reference"=w295) -> ("error out"=w300:errorcluster)  [unwired: 9 in]
        n118 = Compound Arithmetic op=AND(invert w300, w297, invert w289, w298, w285) -> (w310:bool)
        n119 = case shown="True" w310 {
          tunnel: w314 -> [w318 w319]
          tunnel: [w315 w319] -> w313
          tunnel: "Failed lossy fifo pubsub" -> [w317 _]
          tunnel: "\r" -> [w316 _]
          frame False {
            n120 = Concatenate Strings(w318, w317, w316) -> (w315:string)
          }
          frame True {
          }
        }
      }
      frame 9 {
        w326 = T2 {"Name"="Name", "Topic"="Topic", "Type"="", "Best Effort Subscribers"=1, "Backpressure Subscribers"=0, "Best Effort Queue Depth"=1, "Backpressure Queue Depth"=0} ("Publisher Configuration")
        # "Get Publisher Info"
        n121 = call "Initialize.vi"("error in (no error)"=w333, "Node name"="my_node") -> ("error out"=w331:errorcluster)  [unwired: 9 in]
        n122 = call "Create Publisher.vim"("error in (no error)"=w331, "Data"=0.0, "Publisher Configuration"=w326) -> ("error out"=w322:errorcluster, "Publisher Reference"=w330:T4)  [unwired: 6 in, 1 out]
        n123 = Unbundle By Name(w326) -> ("Name"=w325:string, "Topic"=w324:string)
        n124 = call "Read Publisher Info.vi"("error in (no error)"=w322, "Topic"=w324, "Name"=w325) -> ("error out"=w321:errorcluster, "Publisher Info"=w323:T3)  [unwired: 7 in]
        n125 = Equal?(x=w323, y=T3 {"Type"="f64", "Element Size"=8, "Max Elements in Array"=1, "Backpressure Queue Depth"=0, "Best Effort Queue Depth"=1} ("Publisher Info")) -> (x = y?=w327:bool)
        n126 = call "Destroy Publisher.vi"("error in (no error)"=w321, "Publisher Reference"=w330) -> ("error out"=w329:errorcluster)  [unwired: 9 in]
        n127 = Compound Arithmetic op=AND(invert w329, w327) -> (w334:bool)
        n128 = case shown="True" w334 {
          tunnel: w338 -> [w342 w343]
          tunnel: [w339 w343] -> w337
          tunnel: "Failed get publisher info" -> [w341 _]
          tunnel: "\r" -> [w340 _]
          frame False {
            n129 = Concatenate Strings(w342, w341, w340) -> (w339:string)
          }
          frame True {
          }
        }
      }
    }
  }
  "error out" <- w1
  "status" <- w3
  n130 = And Array Elements(Boolean array=w7) -> (logical AND=→"pass":bool)
